vi "ZM-ROOT-launchCm.vi"(8 "error in (no error)":errorcluster, 11 "ZM-ROOT-root in":refnum<class "ZM-ROOT-root.lvclass">) -> (0 "error out":errorcluster, 3 "ZM-ROOT-root out":refnum<class "ZM-ROOT-root.lvclass">)   [LabVIEW 2020, in "ZM-ROOT-root.lvlib" / "ZM-ROOT-root.lvclass"]
doc: "Launches the communication manager, called by ZM-ROOT-init before launchHwm. Its protocol is a multi protocol holding a file logger (writing to the root's outputFolder) and a UDP sender with its defaults. Stores its enqueuer and sets cmRunning = TRUE."
uses:
  ZM-ROOT-root.lvclass
  protocol/ZM-CP-FL-file_logger/ZM-CP-FL-file_logger/ZM-CP-FL-file_logger.lvclass
  protocol/ZM-CP-UDP-udp_transport/ZM-CP-UDP-sender/ZM-CP-UDP-sender.lvclass
  protocol/ZM-CP-communication_protocol/ZM-CP-communication_protocol/ZM-CP-communication_protocol.lvclass
  protocol/ZM-CP-MX-multi_protocol/ZM-CP-MX-multi_protocol/ZM-CP-MX-multi_protocol.lvclass
  ZM-ROOT-root.lvclass/ZM-ROOT-root.ctl
  ZM-CM-communication_manager/ZM-CM-communication_manager/ZM-CM-communication_manager.lvclass
  <vilib>/ActorFramework/Actor/Actor.lvclass
  ZM-CM-communication_manager/ZM-CM-communication_manager/ZM-CM-PRELAUNCH_SETTINGS.ctl
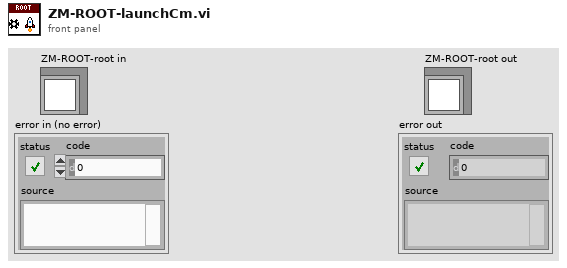
[diagram p1: front panel]
types:
  T1 = typedef "ZM-CM-communication_manager.lvlib/ZM-CM-communication_manager.lvclass/ZM-CM-PRELAUNCH_SETTINGS.ctl" = cluster{"protocol":refnum<class "ZM-CP-communication_protocol.lvclass">}
  T2 = typedef "ZM-ROOT-root.lvlib/ZM-ROOT-root.lvclass/ZM-ROOT-PRELAUNCH_SETTINGS.ctl" = cluster{"outputFolder":path, "usePlaceholderHardware":bool}
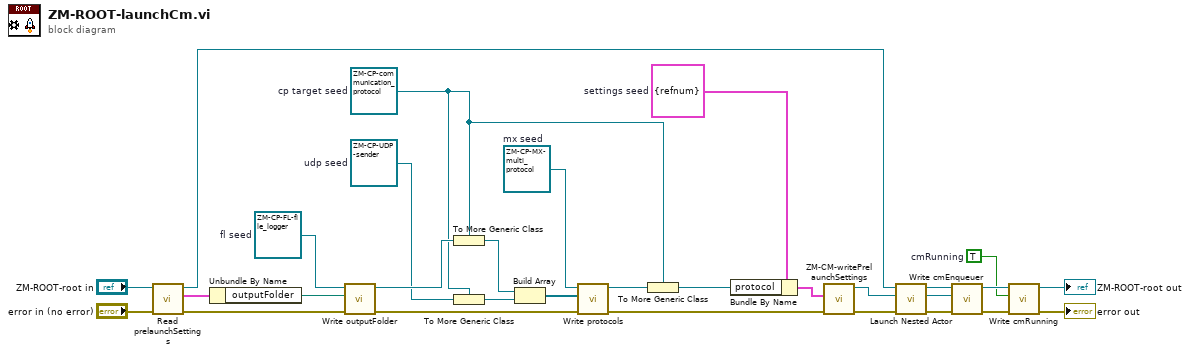
[diagram p0: block diagram]
diagram:
  w3 = TRUE  # cmRunning
  w14 = T1 {"protocol"=refnum}  # settings seed
  w20 = refnum<class "ZM-CP-MX-multi_protocol.lvclass"> refnum  # mx seed
  w16 = refnum<class "ZM-CP-communication_protocol.lvclass"> refnum  # cp target seed
  w23 = refnum<class "ZM-CP-UDP-sender.lvclass"> refnum  # udp seed
  w26 = refnum<class "ZM-CP-FL-file_logger.lvclass"> refnum  # fl seed
  n1 = call "Read prelaunchSettings.vi"("error in (no error)"="error in (no error)", "ZM-ROOT-root in"="ZM-ROOT-root in") -> ("error out"=w27:errorcluster, "ZM-ROOT-PRELAUNCH_SETTINGS"=w28:T2, "ZM-ROOT-root out"=w9:refnum<class "ZM-ROOT-root.lvclass">)  [unwired: 7 in]
  n2 = Unbundle By Name(w28) -> ("outputFolder"=w25:path)
  n3 = call "Write outputFolder.vi"("error in (no error)"=w27, "outputFolder"=w25, "ZM-CP-FL-file_logger in"=w26) -> ("error out"=w18:errorcluster, "ZM-CP-FL-file_logger out"=w24:refnum<class "ZM-CP-FL-file_logger.lvclass">)  [unwired: 7 in]
  n4 = To More Generic Class(target class=w16, reference=w24) -> (generic class reference=w22:refnum<class "ZM-CP-communication_protocol.lvclass">)
  n5 = To More Generic Class(target class=w16, reference=w23) -> (generic class reference=w21:refnum<class "ZM-CP-communication_protocol.lvclass">)
  n6 = Build Array(w22, w21) -> (w19:refnum<class "ZM-CP-communication_protocol.lvclass">[])
  n7 = call "Write protocols.vi"("error in (no error)"=w18, "ZM-CP-MX-PROTOCOLS"=w19, "ZM-CP-MX-multi_protocol in"=w20) -> ("error out"=w12:errorcluster, "ZM-CP-MX-multi_protocol out"=w17:refnum<class "ZM-CP-MX-multi_protocol.lvclass">)  [unwired: 7 in]
  n8 = To More Generic Class(target class=w16, reference=w17) -> (generic class reference=w15:refnum<class "ZM-CP-communication_protocol.lvclass">)
  n9 = Bundle By Name(cluster=w14, "protocol"=w15) -> (w13:T1)
  n10 = call "ZM-CM-writePrelaunchSettings.vi"("error in (no error)"=w12, "settings"=w13) -> ("error out"=w10:errorcluster, "ZM-CM-communication_manager out"=w11:refnum<class "ZM-CM-communication_manager.lvclass">)  [unwired: 8 in]
  n11 = call <vilib>:"Launch Nested Actor.vi"("error in (no error)"=w10, "Nested Actor"=w11, "Caller Actor in"=w9) -> ("error out"=w8:errorcluster, "Nested Actor's Enqueuer"=w6:refnum<class "Message Enqueuer.lvclass">, "Caller Actor out"=w7:refnum<class "ZM-ROOT-root.lvclass">)  [unwired: 6 in]
  n12 = call "Write cmEnqueuer.vi"("error in (no error)"=w8, "Actor Framework:Message Enqueuer"=w6, "ZM-ROOT-root in"=w7) -> ("error out"=w5:errorcluster, "ZM-ROOT-root out"=w4:refnum<class "ZM-ROOT-root.lvclass">)  [unwired: 7 in]
  n13 = call "Write cmRunning.vi"("error in (no error)"=w5, "cmRunning"=w3, "ZM-ROOT-root in"=w4) -> ("error out"=→"error out":errorcluster, "ZM-ROOT-root out"=→"ZM-ROOT-root out":refnum<class "ZM-ROOT-root.lvclass">)  [unwired: 7 in]
